vi "Update Setpoint Typedef.vi"(10 "VI Refs":refnum<vi>[](array[refnum]), 11 "Subsystem Name":string) -> (0 "error out":errorcluster)   [LabVIEW 2023]
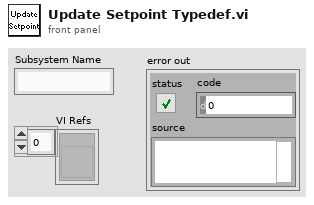
[diagram p1: front panel]
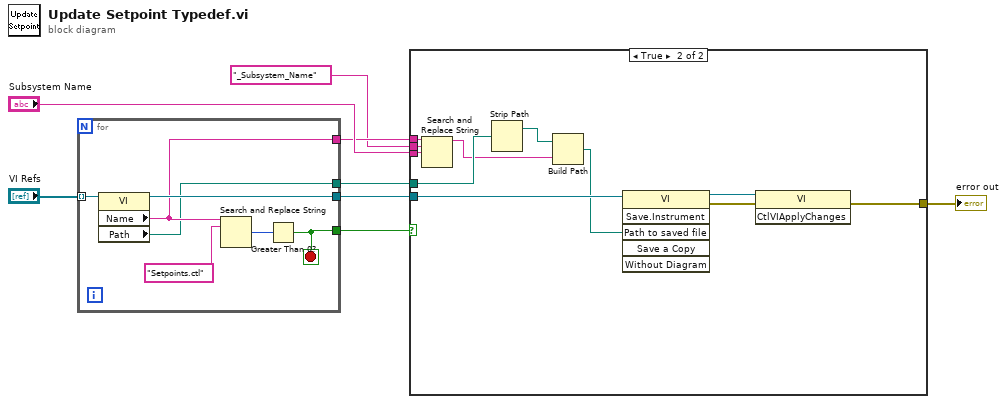
[diagram p0: block diagram]
diagram:
  n1 = for {
    tunnel: "VI Refs" -> [w13] mode=indexing
    tunnel: [w9] -> w1
    tunnel: [w12] -> w5
    tunnel: [w11] -> w3
    tunnel: [w10] -> w4
    stop <- w9 stop-if-true
    n2 = property class="VI"(reference=w13) -> (reference out=w12:refnum<vi>, "Name"=w11:string, "Path"=w10:path)  [unwired: 1 in, 1 out]
    n3 = Search and Replace String(input string=w11, search string="Setpoints.ctl") -> (number of replacements=w14:i32)  [unwired: 6 in, 3 out]
    n4 = Greater Than 0?(x=w14) -> (x > 0?=w9:bool)
  }
  n5 = case shown="True" w1 {
    tunnel: "Subsystem Name" -> [_ w26]
    tunnel: [_ w25] -> w7
    tunnel: w5 -> [_ w24]
    tunnel: w4 -> [_ w22]
    tunnel: w3 -> [_ w21]
    tunnel: "_Subsystem_Name" -> [_ w20]
    frame False {
    }
    frame True {
      n6 = Search and Replace String(input string=w21, search string=w20, replace string=w26) -> (result string=w19:string)  [unwired: 5 in, 3 out]
      n7 = Strip Path(path=w22) -> (stripped path=w18:path)  [unwired: 1 out]
      n8 = Build Path(base path=w18, name or relative path=w19) -> (appended path=w23:path)
      n9 = invoke class="VI" method="Save.Instrument"(reference=w24, "Path to saved file"=w23) -> (reference out=w17:refnum<vi>, error out=w16:errorcluster)  [unwired: 4 in, 4 out]
      n10 = invoke class="VI" method="CtlVIApplyChanges"(reference=w17, error in=w16) -> (error out=w25:errorcluster)  [unwired: 1 in, 2 out]
    }
  }
  "error out" <- w7
